vi "move files to target folder.vi"(8 "error in":errorcluster, 9 "overwrite (F)":bool, 10 "files":path[](array[path])=[path "C:/Users/Benjamin/Desktop/Test Folders/Folder odd/file 1.txt", path "C:/Users/Benjamin/Desktop/Test Folders/Folder odd/file 3.txt", path "C:/Users/Benjamin/Desktop/Test Folders/Folder odd/file 5.txt", path "C:/Users/Benjamin/Desktop/Test Folders/Folder odd/file 7.txt"], 11 "target folder":path=path "C:/Users/Benjamin/Desktop/Destination Folder") -> (0 "error out":errorcluster, 2 "new file paths":path[](array[path]), 3 "target folder duplicate":path)   [LabVIEW 2014]
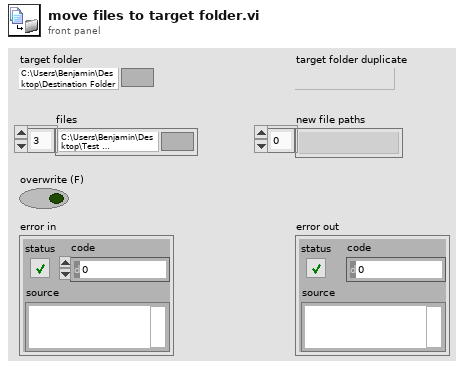
[diagram p1: front panel]
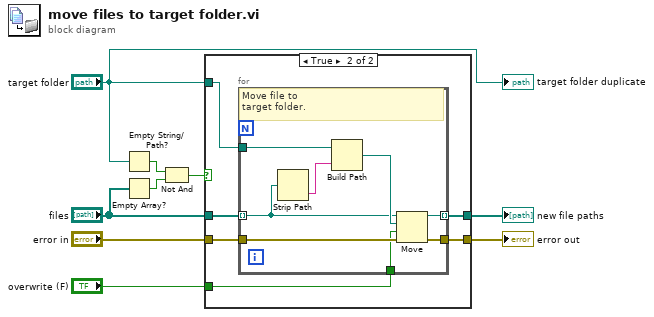
[diagram p0: block diagram]
diagram:
  n1 = Empty String/Path?(string/path="target folder") -> (empty?=w2:bool)
  n2 = Empty Array?(array="files") -> (empty?=w3:bool)
  n3 = Not And(1:w3, 2:w2) -> (0:w1:bool)
  n4 = case shown="True" w1 {
    tunnel: [w10 w17] -> w9
    tunnel: "overwrite (F)" -> [_ w16]
    tunnel: [w11 w15] -> w7
    tunnel: "error in" -> [w10 w14]
    tunnel: "target folder" -> [_ w13]
    tunnel: "files" -> [w11 w12]
    frame False {
      # "Target folder missing OR\nfiles to move are missing."
    }
    frame True {
      n5 = for {
        tunnel: w12 -> [w19] mode=indexing
        tunnel: w13 -> [w25]
        tunnel: w14 -> [w23]
        tunnel: [w22] -> w17
        tunnel: w16 -> [w21]
        tunnel: [w20] -> w15 mode=indexing
        # "Move file to \ntarget folder."
        n6 = Strip Path(path=w19) -> (name=w18:string)  [unwired: 1 out]
        n7 = Build Path(base path=w25, name or relative path=w18) -> (appended path=w24:path)
        n8 = Move(source path=w19, error in=w23, 9:w21, 10:w24) -> (error out=w22:errorcluster, 3:w20:path)  [unwired: 1 in, 1 out]
      }
    }
  }
  "error out" <- w9
  "new file paths" <- w7
  "target folder duplicate" <- "target folder"
